vi "Test_Column.vi"(10 "Enum":T1, 11 "Enum":T2) -> (3 "Enum":T2)   [LabVIEW 2021]
uses:
  FGI.ctl
  Get_Set.ctl
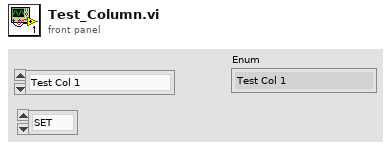
[diagram p1: front panel]
types:
  T1 = typedef "Get_Set.ctl" = enum16{"SET", "GET"}
  T2 = typedef "FGI.ctl" = enum16{"Test Col 1", "Test Col 2"}
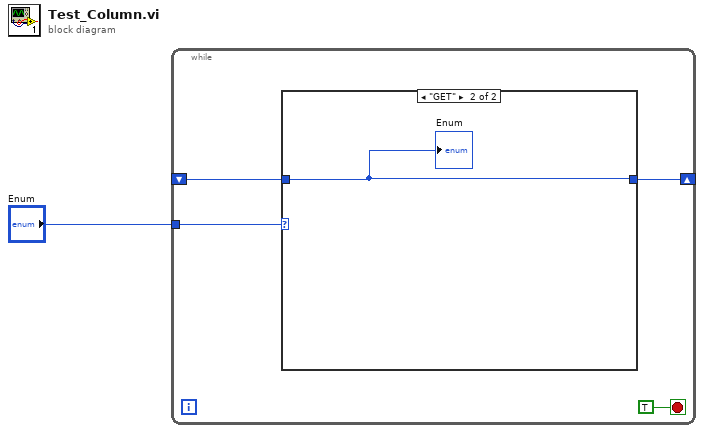
[diagram p0: block diagram]
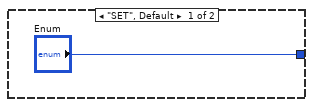
[diagram p2: hidden frame]
diagram:
  n1 = while {
    tunnel: "Enum" -> [w5]
    shift-right: [w4] -> _
    shift-left: _ -> [w3]
    stop <- TRUE stop-if-true
    n2 = case shown="\"GET\"" w5 {
      tunnel: ["Enum" w7] -> w4
      tunnel: w3 -> [_ w7]
      frame "SET", Default {
      }
      frame "GET" {
        "Enum" <- w7
      }
    }
  }
